vi "Read sound from a file.vi"(8 "error in":errorcluster, 11 "path":path) -> (0 "error out":errorcluster, 2 "rate out":enum16{"11025", "22050", "44100"}(ring), 3 "Data (mono)":dbl[](array[numeric]))   [LabVIEW 2021]
doc: "::: CalcExpress Toolkit :::\nCopyright (c) 2000-2026 Konstantin Shifershteyn. All rights reserved."
uses:
  <vilib>/sound2/lvsound2.llb/Sound Data Format.ctl
  <vilib>/Analysis/baseanly.llb/Mean (DBL).vi
  <vilib>/sound2/lvsound2.llb/Sound File Read Open.vi
  <vilib>/sound2/lvsound2.llb/Sound File Info (refnum).vi
  <vilib>/sound2/lvsound2.llb/Sound File Read (DBL).vi
  <vilib>/Analysis/NI_AALBase.lvlib
panel:
  out "sound format":T1={"sample rate (S/s)"=22050.0, "number of channels"=2, "bits per sample"=16}
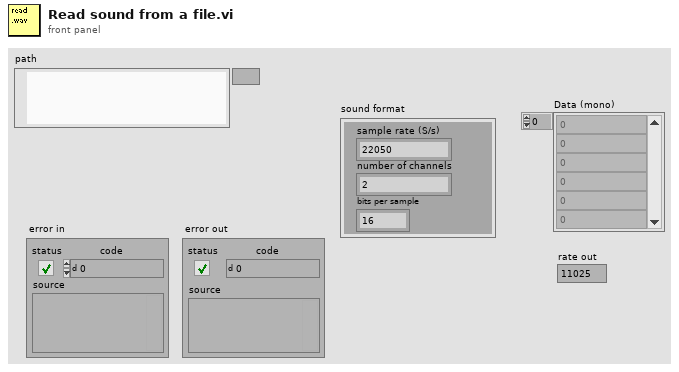
[diagram p1: front panel]
types:
  T1 = typedef "Sound Data Format.ctl" = cluster{"sample rate (S/s)":dbl, "number of channels":i32, "bits per sample":i32}
  T2 = typedef "Sound File Refnum.ctl" = refnum<file>
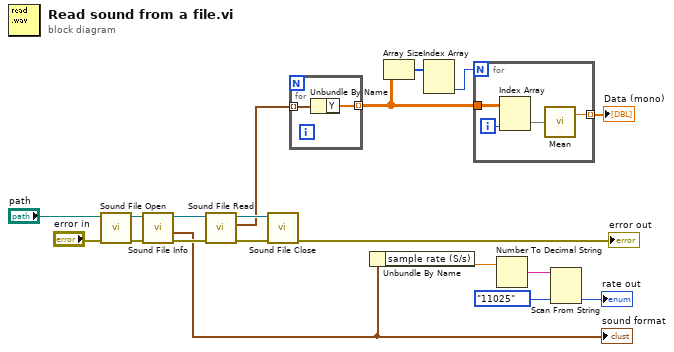
[diagram p0: block diagram]
diagram:
  n1 = call-poly <vilib>:"Sound File Open.vi"("error in (no error)"="error in", "path"="path") -> ("error out"=w17:errorcluster, "sound file refnum"=w19:T2)  [unwired: 8 in]
  n2 = call-poly <vilib>:"Sound File Info.vi"("error in (no error)"=w17, "sound file refnum"=w19) -> ("error out"=w15:errorcluster, "sound format"=w5:T1, "sound file refnum out"=w16:T2)  [unwired: 6 in, 1 out]
  "sound format" <- w5
  n3 = call-poly <vilib>:"Sound File Read.vi"("error in (no error)"=w15, "sound file refnum"=w16) -> ("error out"=w13:errorcluster, "data"=w12:waveform(dbl)[], "sound file refnum out"=w14:T2)  [unwired: 5 in, 2 out]
  n4 = call <vilib>:"Sound File Close.vi"("error in (no error)"=w13, "sound file refnum"=w14) -> ("error out"=→"error out":errorcluster)  [unwired: 9 in]
  n5 = for {
    tunnel: [w21] -> w10 mode=indexing
    tunnel: w12 -> [w20] mode=indexing
    n6 = Unbundle By Name(w20) -> ("Y"=w21:dbl[])
  }
  n7 = Unbundle By Name(w5) -> ("sample rate (S/s)"=w4:dbl)
  n8 = Array Size(array=w10) -> (size(s)=w11:i32[])
  n9 = Index Array(array=w11) -> (element #2=w9:i32)  [unwired: 2 in, 1 out]
  n10 = for {
    N: w9 -> [_]
    tunnel: w10 -> [w25]
    tunnel: [w22] -> w8 mode=indexing
    i -> [w24]
    n11 = Index Array(array=w25, index (col)=w24) -> (element=w23:dbl[])  [unwired: 1 in]
    n12 = call-poly <vilib>:"Mean.vi"("X"=w23) -> ("mean"=w22:dbl)  [unwired: 1 out]
  }
  "Data (mono)" <- w8
  n13 = Number To Decimal String(number=w4) -> (decimal integer string=w3:string)  [unwired: 1 in]
  n14 = Scan From String(input string=w3, default 1=enum16{"11025", "22050", "44100"}."11025" ("rate out")) -> (output 1=→"rate out":enum16{"11025", "22050", "44100"})  [unwired: 3 in, 3 out]
